vi "Remove Empty Description.vi"(11 "schema":string) -> (3 "schema out":string)   [LabVIEW 2020, in "MCP Server.lvlib"]
doc: "Returns the JSON object schema without its \"description\" item when that item is an empty string. A description key without text tells an MCP client nothing, so tools/list leaves it out of an input's schema - whether the input had no description to begin with or Remove Default Error Description.vi emptied it. Every other item is kept in its order, and an object without an empty description is returned unchanged, character for character. Text that is not a JSON object is returned unchanged."
uses:
  MCP Server.lvlib
  <vilib>/JDP Science/JSONtext/support/Format JSON Object.vi
  <vilib>/JDP Science/JSONtext/JSONtext.lvlib
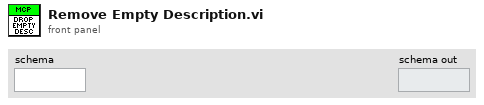
[diagram p1: front panel]
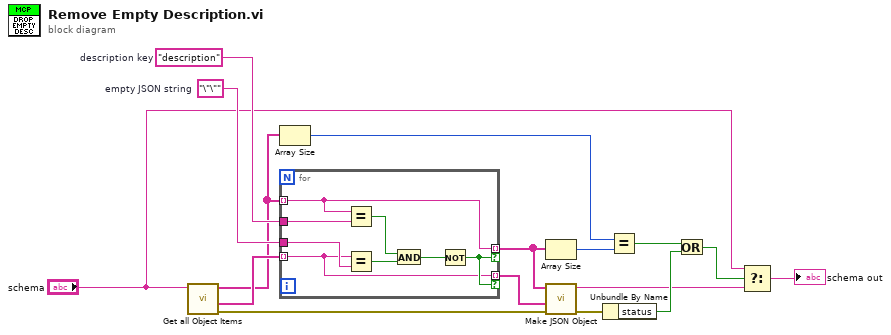
[diagram p0: block diagram]
diagram:
  w14 = "\"\""  # empty JSON string
  w15 = "description"  # description key
  n1 = call <vilib>:"Get all Object Items.vi"("JSON"="schema") -> ("error out"=w12:errorcluster, "<JSON>"=w16:string[], "Item Names"=w11:string[])  [unwired: 7 in, 1 out]
  n2 = Array Size(array=w11) -> (size(s)=w9:i32)
  n3 = for {
    tunnel: w11 -> [w19] mode=indexing
    tunnel: w16 -> [w17] mode=indexing
    tunnel: w15 -> [w24]
    tunnel: w14 -> [w23]
    tunnel: [w19] -> w10 mode=indexing if=w18
    tunnel: [w17] -> w13 mode=indexing if=w18
    n4 = Equal?(x=w19, y=w24) -> (x = y?=w22:bool)
    n5 = Equal?(x=w17, y=w23) -> (x = y?=w21:bool)
    n6 = And(x=w22, y=w21) -> (x .and. y?=w20:bool)
    n7 = Not(x=w20) -> (.not. x?=w18:bool)
  }
  n8 = Array Size(array=w10) -> (size(s)=w8:i32)
  n9 = call <vilib>:"Make JSON Object.vi"("error in (no error)"=w12, "JSON Items"=w13, "Item Names"=w10) -> ("error out"=w7:errorcluster, "<JSON>"=w2:string)  [unwired: 7 in]
  n10 = Unbundle By Name(w7) -> ("status"=w5:bool)
  n11 = Equal?(x=w9, y=w8) -> (x = y?=w6:bool)
  n12 = Or(x=w6, y=w5) -> (x .or. y?=w3:bool)
  n13 = Select(t="schema", s=w3, f=w2) -> (s? t:f=→"schema out":string)
